vi "Get Library Info.vi"(8 "error in (no error)":errorcluster) -> (0 "error out":errorcluster, 1 "License":string, 2 "Copyright":string, 3 "Version String":string, 5 "Name":string)   [LabVIEW 2020, in "Caraya.lvlib"]
uses:
  Caraya.lvlib
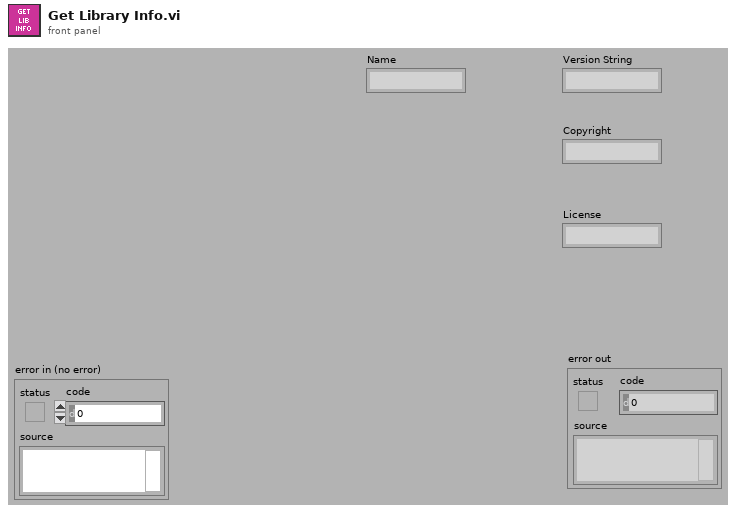
[diagram p1: front panel]
types:
  T1 = cluster{"Version String":string, "Name":string, "Copyright":string, "License":string}
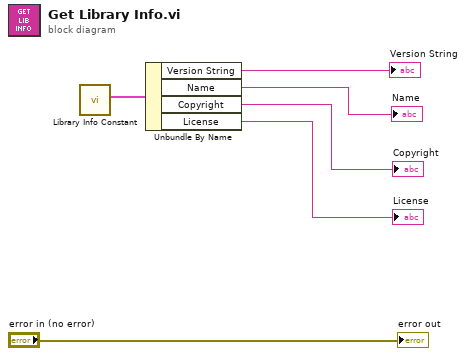
[diagram p0: block diagram]
diagram:
  n1 = call "Library Info Constant.vi"() -> ("Library Info Constant"=w5:T1)  [unwired: 11 in]
  n2 = Unbundle By Name(w5) -> ("Version String"=→"Version String":string, "Name"=→"Name":string, "Copyright"=→"Copyright":string, "License"=→"License":string)
  "error out" <- "error in (no error)"
